vi "IOMenu.vi"(0 "ip":string) -> ()   [LabVIEW 2024]
panel:
  in  "Switch":bool
  in  "Cancel Button":bool
  in  "OK Button":bool
  # "OLED Screen Setting Menu"
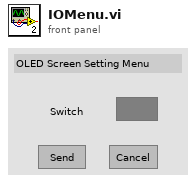
[diagram p1: front panel]
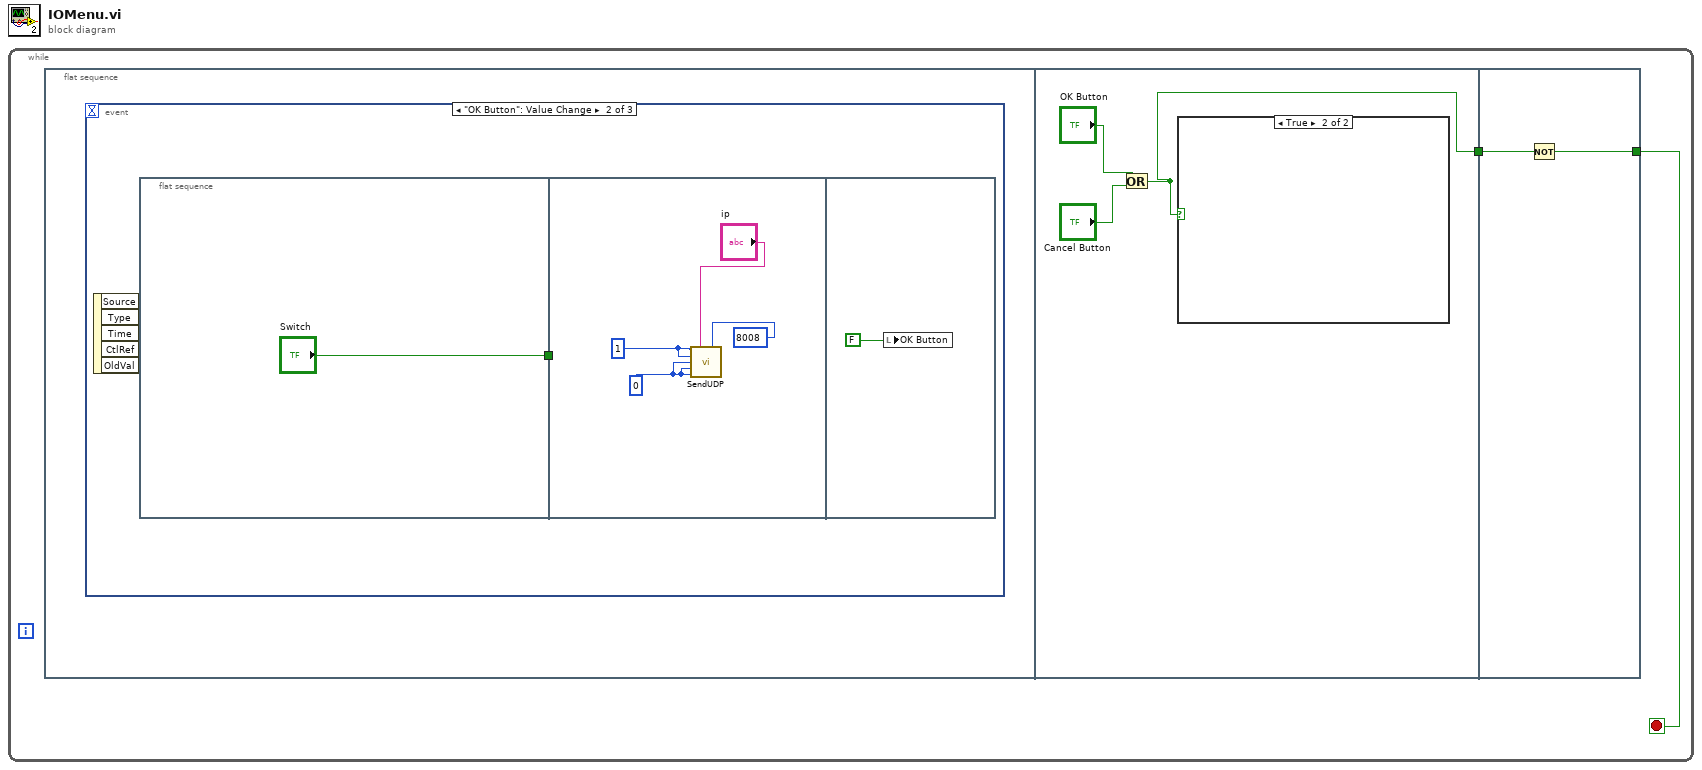
[diagram p0: block diagram]
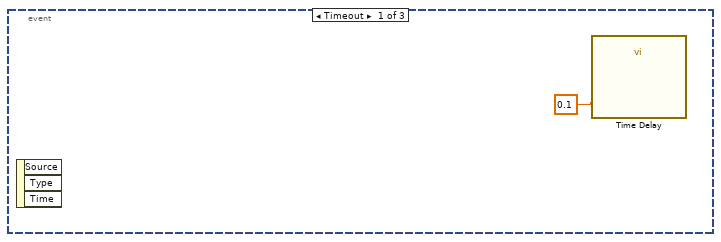
[diagram p2: hidden frame]
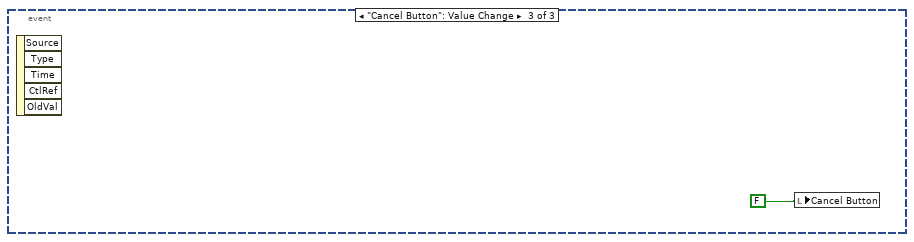
[diagram p3: hidden frame]
diagram:
  n1 = while {
    stop <- w2 stop-if-true
    n2 = flat-sequence {
      tunnel: [w12] -> w1
      tunnel: [w16] -> w2
      tunnel: w1 -> [w15]
      frame #0 {
        n3 = event shown="[1] \"OK Button\": Value Change" {
          selector: _ -> [_ _ _]
          dyn-events: _ -> [_ _ _]
          timeout: _ -> [_ _ _]
          event Timeout {
            n4 = event-data() -> ()  [unwired: 1 in, 3 out]
            n5 = call "Time Delay"("Delay Time (s)"=0.1) -> ()  [unwired: 10 in, 1 out]
          }
          event "OK Button": Value Change {
            n6 = event-data() -> ()  [unwired: 1 in, 5 out]
            n7 = flat-sequence {
              tunnel: ["Switch"] -> w4
              tunnel: w4 -> [_]
              frame #0 {
              }
              frame #1 {
                w6 = u8 1 ("Arg3")
                w7 = u8 0 ("Arg7")
                n8 = call "SendUDP.vi"("Arg3"=w6, "IP"="ip", "Port"=8008, "Arg4"=w6, "Arg5"=w7, "Arg6"=w7, "Arg7"=w7) -> ()  [unwired: 9 in]
              }
              frame #2 {
                n9 = local write "OK Button"(FALSE ("OK Button")) -> ()
              }
            }
          }
          event "Cancel Button": Value Change {
            n10 = event-data() -> ()  [unwired: 1 in, 5 out]
            n11 = local write "Cancel Button"(FALSE ("Cancel Button")) -> ()
          }
        }
      }
      frame #1 {
        n12 = Or(x="OK Button", y="Cancel Button") -> (x .or. y?=w12:bool)
        n13 = case shown="True" w12 {
          frame False {
          }
          frame True {
          }
        }
      }
      frame #2 {
        n14 = Not(x=w15) -> (.not. x?=w16:bool)
      }
    }
  }
